vi "Open In Project.vi"(0 "project path":string, 5 "vi paths":string, 7 "show front panels":bool=TRUE, 11 "error in":errorcluster) -> (4 "opened":i32, 6 "report":string, 15 "error out":errorcluster)   [LabVIEW 2026]
doc: "Opens a LabVIEW project and then opens VIs FROM it, the way a user double-clicks them in the Project Explorer. Project.Open loads the project (an already-open one is reused) and Open Window shows it. For each path in vi paths (separated by ;, in order) the VI is looked up among the project's VI items (Dependencies included) by file path (case-insensitive), opened with Open VI Reference on the application instance of the project's My Computer target, and - if show front panels is true - its front panel is opened with FP.Open so LabVIEW fully loads and compiles it. A VI that fails does not stop the others. The project and the opened panels stay open when this VI finishes; only the references are closed. With show front panels false LabVIEW may unload the VIs again once this VI goes idle. report has one line per VI: '<path> -> ok' or '<path> -> error <code>: <source>'. A VI that is not an item of the project gives error 5000. error out carries the first error of the whole run, project or VI. Done goes true last, after every other indicator is written."
uses:
  <vilib>/AdvancedString/Delimited String to 1D String Array (string).vi
panel:
  out "Done":bool
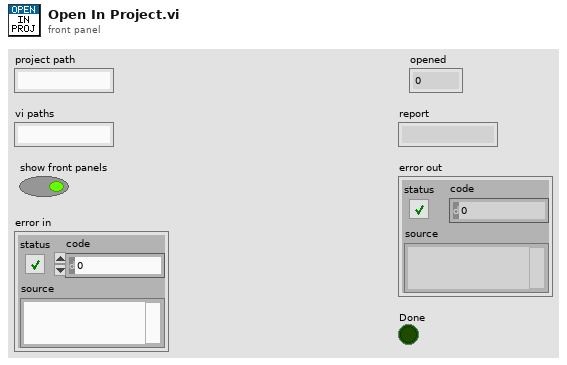
[diagram p1: front panel]
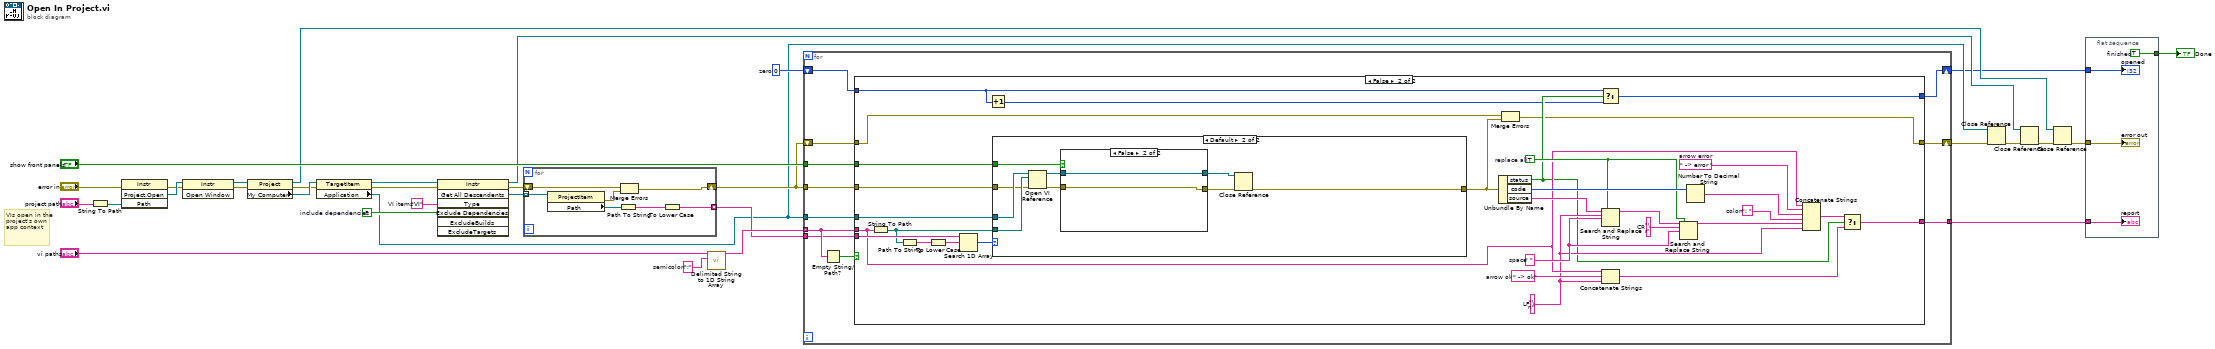
[diagram p0: block diagram]
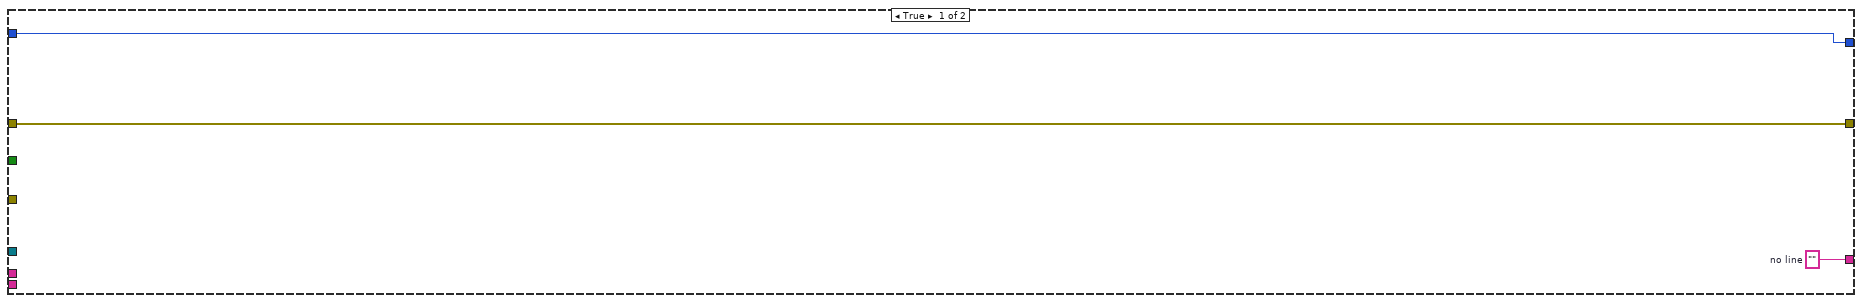
[diagram p2: hidden frame]
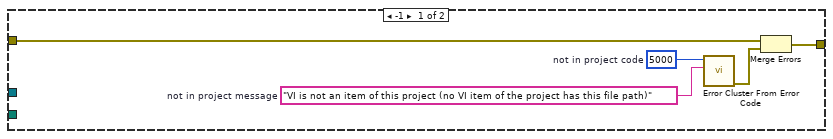
[diagram p3: hidden frame]
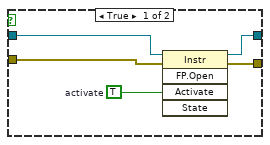
[diagram p4: hidden frame]
diagram:
  w12 = 0  # zero
  w20 = FALSE  # include dependencies
  w21 = "VI"  # VI items
  w16 = ";"  # semicolon
  # "VIs open in the project's own app context"
  n1 = String To Path(string="project path") -> (path=w30:path)
  n2 = invoke class="Instr" method="Project.Open"(error in="error in", "Path"=w30) -> (error out=w28:errorcluster, "Project:Open"=w29:refnum<vi>)  [unwired: 2 in, 2 out]
  n3 = invoke class="Instr" method="Open Window"(reference=w29, error in=w28) -> (reference out=w27:refnum<vi>, error out=w26:errorcluster)  [unwired: 1 in, 1 out]
  n4 = property class="Project"(reference=w27, error in=w26) -> (reference out=w6:refnum<vi>, error out=w24:errorcluster, "My Computer"=w25:refnum<vi>)
  n5 = property class="TargetItem"(reference=w25, error in=w24) -> (reference out=w23:refnum<vi>, error out=w22:errorcluster, "Application"=w10:refnum<vi>)
  n6 = invoke class="Instr" method="Get All Descendents"(reference=w23, error in=w22, "Type"=w21, "Exclude Dependencies"=w20) -> (reference out=w8:refnum<vi>, error out=w18:errorcluster, "All Descendents"=w19:refnum<vi>[])  [unwired: 3 in, 4 out]
  n7 = for {
    tunnel: w19 -> [w39] mode=indexing
    tunnel: [w35] -> w14 mode=indexing
    shift-right: [w34] -> w11
    shift-left: w18 -> [w33]
    n8 = property class="ProjectItem"(reference=w39) -> (error out=w36:errorcluster, "Path"=w38:path)  [unwired: 1 in, 1 out]
    n9 = Path To String(path=w38) -> (string=w37:string)
    n10 = Merge Errors(w33, w36) -> (w34:errorcluster)
    n11 = To Lower Case(string=w37) -> (all lower case string=w35:string)
  }
  n12 = call-poly <vilib>:"Delimited String to 1D String Array.vi"("delimiter"=w16, "delimited string"="vi paths") -> ("string array"=w15:string[])  [unwired: 9 in]
  n13 = for {
    tunnel: w15 -> [w50] mode=indexing
    tunnel: w14 -> [w49]
    tunnel: w10 -> [w48]
    tunnel: "show front panels" -> [w47]
    tunnel: w11 -> [w46]
    tunnel: [w44] -> w3 mode=concatenating
    shift-right: [w43] -> w4
    shift-left: w12 -> [w42]
    shift-right: [w41] -> w9
    shift-left: w11 -> [w40]
    n14 = Empty String/Path?(string/path=w50) -> (empty?=w45:bool)
    n15 = case shown="False" w45 {
      tunnel: w50 -> [_ w66]
      tunnel: w49 -> [_ w83]
      tunnel: w48 -> [_ w80]
      tunnel: w47 -> [_ w79]
      tunnel: w46 -> [_ w78]
      tunnel: w42 -> [w52 w61]
      tunnel: w40 -> [w51 w58]
      tunnel: [w53 w56] -> w44
      tunnel: [w52 w55] -> w43
      tunnel: [w51 w54] -> w41
      frame True {
        w53 = ""  # no line
      }
      frame False {
        w65 = " -> ok"  # arrow ok
        w68 = ": "  # colon
        w70 = " -> error "  # arrow error
        w71 = TRUE  # replace all
        w72 = " "  # space
        w73 = "\r"  # CR
        w64 = "\n"  # LF
        n16 = String To Path(string=w66) -> (path=w81:path)
        n17 = Path To String(path=w81) -> (string=w84:string)
        n18 = To Lower Case(string=w84) -> (all lower case string=w82:string)
        n19 = Search 1D Array(1D array=w83, element=w82) -> (index of element=w77:i32)  [unwired: 1 in]
        n20 = Increment(x=w61) -> (x+1=w59:i32)
        n21 = case shown="Default" w77 {
          tunnel: w81 -> [_ w97]
          tunnel: w80 -> [_ w98]
          tunnel: w79 -> [_ w93]
          tunnel: w78 -> [w87 w96]
          tunnel: [w85 w90] -> w57
          frame -1 {
            w88 = "VI is not an item of this project (no VI item of the project has this file path)"  # not in project message
            w89 = 5000  # not in project code
            n22 = call <vilib>:"Error Cluster From Error Code.vi"("error message (\"\")"=w88, "error code (0)"=w89) -> ("error out"=w86:errorcluster)  [unwired: 7 in]
            n23 = Merge Errors(w87, w86) -> (w85:errorcluster)
          }
          frame Default {
            n24 = Open VI Reference(application reference (local)=w98, vi path=w97, error in (no error)=w96) -> (vi reference=w95:refnum<vi>, error out=w94:errorcluster)  [unwired: 3 in]
            n25 = case shown="False" w93 {
              tunnel: w95 -> [w103 w105]
              tunnel: w94 -> [w102 w104]
              tunnel: [w100 w105] -> w92
              tunnel: [w99 w104] -> w91
              frame True {
                w101 = TRUE  # activate
                n26 = invoke class="Instr" method="FP.Open"(reference=w103, error in=w102, "Activate"=w101) -> (reference out=w100:refnum<vi>, error out=w99:errorcluster)  [unwired: 2 in, 3 out]
              }
              frame False {
              }
            }
            n27 = Close Reference(reference=w92, error in (no error)=w91) -> (error out=w90:errorcluster)
          }
        }
        n28 = Unbundle By Name(w57) -> ("status"=w60:bool, "code"=w76:i32, "source"=w75:string)
        n29 = Merge Errors(w58, w57) -> (w54:errorcluster)
        n30 = Select(t=w61, s=w60, f=w59) -> (s? t:f=w55:i32)
        n31 = Search and Replace String(replace all?=w71, input string=w75, search string=w64, replace string=w72) -> (result string=w74:string)  [unwired: 4 in, 3 out]
        n32 = Concatenate Strings(w66, w65, w64) -> (w62:string)
        n33 = Search and Replace String(replace all?=w71, input string=w74, search string=w73, replace string=w72) -> (result string=w67:string)  [unwired: 4 in, 3 out]
        n34 = Number To Decimal String(number=w76) -> (decimal integer string=w69:string)  [unwired: 1 in]
        n35 = Concatenate Strings(w66, w70, w69, w68, w67, w64) -> (w63:string)
        n36 = Select(t=w63, s=w60, f=w62) -> (s? t:f=w56:string)
      }
    }
  }
  n37 = Close Reference(reference=w10, error in (no error)=w9) -> (error out=w7:errorcluster)
  n38 = Close Reference(reference=w8, error in (no error)=w7) -> (error out=w5:errorcluster)
  n39 = Close Reference(reference=w6, error in (no error)=w5) -> (error out=w2:errorcluster)
  n40 = flat-sequence {
    tunnel: w4 -> [w109]
    tunnel: w3 -> [w108]
    tunnel: w2 -> [w107]
    tunnel: [w106] -> w1
    frame #0 {
      w106 = TRUE  # finished
      "opened" <- w109
      "report" <- w108
      "error out" <- w107
    }
  }
  "Done" <- w1
